vi "Missing VI Message.vi"() -> ()   [LabVIEW 2020, in "Peek Window.lvlib" / "Missing VI Type.lvclass"]
uses:
  Missing VI Type.lvclass
panel:
  out "VI Path":path
  out "VI Full Qualified Name":string
  # "This VI is Missing. \nThe Block Diagram cannot be displayed."
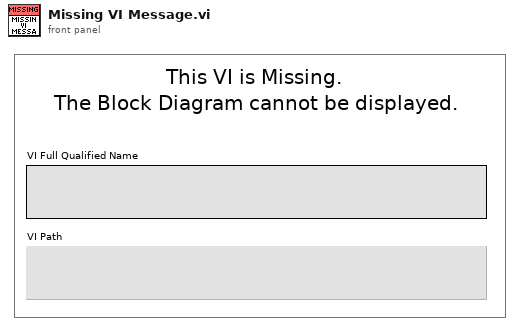
[diagram p1: front panel]
diagram:
